vi "simpleReadWrite.vi"() -> ()   [LabVIEW 2015, in "labOpenShowVar.lvlib"]
uses:
  <vilib>/Platform/TimedLoop/XDataNode/timing_clust.ctl
  <vilib>/Platform/TimedLoop/XDataNode/nitl_modes.ctl
  <vilib>/Platform/TimedLoop/XDataNode/wakeup.ctl
  <vilib>/Platform/TimedLoop/XDataNode/XDataNode.xnode
  labOpenShowVar.lvlib
  <vilib>/Platform/TimedLoop/XDataNode/XDNodeRunTimeDep.lvlib
panel:
  in  "id":u16=1
  in  "写入":bool
  in  "value":string
  out "data":string
  in  "var":string="aaa"
  in  "停止":bool
  in  "ip":string="172.31.1.147"
  # "简单的变量读写"
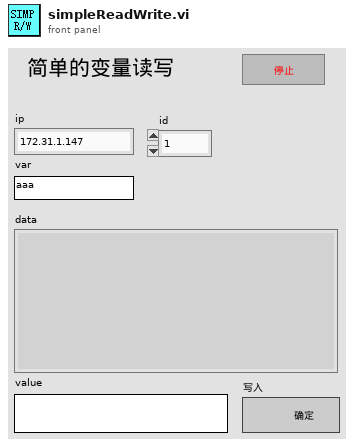
[diagram p1: front panel]
types:
  T1 = typedef "XDNodeRunTimeDep.lvlib/timing_clust.ctl" = cluster{"Expected End [f-1]":u64, "Actual End [f-1]":u64, "Finished Late? [f-1]":bool, "Expected End [i-1]":u64, "Actual End [i-1]":u64, "Finished Late? [i-1]":bool, "Expected Start [i]":u64, "Actual Start [i]":u64, "Expected Start [f]":u64, "Actual Start [f]":u64, "Source Name":string, "Structure Name":string, "Period":i64, "Deadline":i64, "Offset":i64, "Start":i64, "Priority":i32, "Timeout":i32, "Mode":T2, "Wakeup Reason":T3, "Error":errorcluster, "Source Type":string, "Secondary Source Type":string, "Global End Time":u64, "Global Start Time":u64, "Frame Duration":u64, "Iteration Duration":u64, "Assigned CPU":i32, "I/O Scan Engine Mode":u32}
  T2 = typedef "XDNodeRunTimeDep.lvlib/nitl_modes.ctl" = enum32{"No Change", "Process missed periods, maintain original phase", "Discard missed periods, maintain original phase", "Process missed periods, ignore original phase", "Discard missed periods, ignore original phase"}
  T3 = typedef "XDNodeRunTimeDep.lvlib/wakeup.ctl" = enum32{"Normal", "Aborted", "Asynchronous wakeup", "Timing source error", "Timed loop error", "Timeout"}
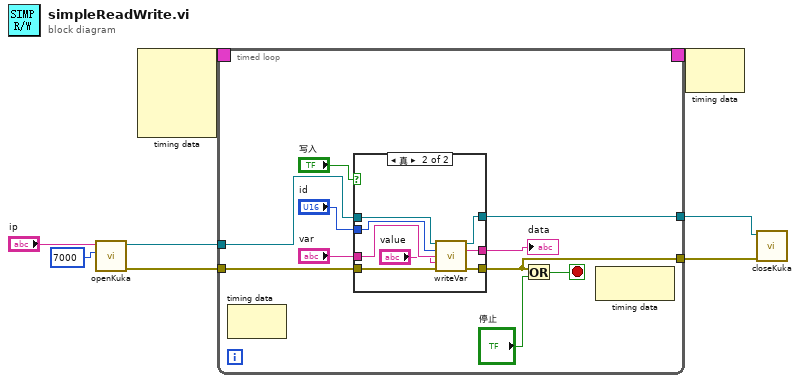
[diagram p0: block diagram]
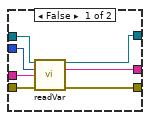
[diagram p2: hidden frame]
diagram:
  n1 = call "openKuka.vi"("远程端口或服务名称"=u16 7000, "地址"="ip") -> ("错误输出"=w5:errorcluster, "TCP网络连接输出"=w6:refnum<k5>)  [unwired: 8 in]
  n2 = node-c288() -> (w4:T1)  [unwired: 4 in]
  n3 = timed-loop {
    tunnel: w6 -> [w15]
    tunnel: w5 -> [w14]
    timing: w4 -> [_]
    timing-out: [_] -> w3
    tunnel: [w13] -> w2
    tunnel: [w10] -> w1
    stop <- w11 stop-if-true
    n4 = node-c288() -> ()  [unwired: 1 in, 1 out]
    n5 = case shown="真" "写入" {
      tunnel: "id" -> [w22 w32]
      tunnel: "var" -> [w21 w31]
      tunnel: w15 -> [w25 w33]
      tunnel: w14 -> [w24 w30]
      tunnel: [w23 w28] -> w13
      tunnel: [w20 w27] -> w10
      tunnel: [w19 w26] -> w9
      frame False {
        n6 = call "readVar.vi"("TCP网络连接输入"=w25, "id"=w22, "var"=w21, "错误输入（无错误）"=w24) -> ("TCP网络连接输出"=w23:refnum<k5>, "data out"=w19:string, "错误输出"=w20:errorcluster)  [unwired: 9 in]
      }
      frame True {
        n7 = call "writeVar.vi"("TCP网络连接输入"=w33, "id"=w32, "var"=w31, "val"="value", "错误输入（无错误）"=w30) -> ("TCP网络连接输出"=w28:refnum<k5>, "data out"=w26:string, "错误输出"=w27:errorcluster)  [unwired: 8 in]
      }
    }
    "data" <- w9
    n8 = Or(x=w10, y="停止") -> (x .or. y?=w11:bool)
    n9 = node-c288() -> ()  [unwired: 1 in, 1 out]
  }
  n10 = node-c288(w3) -> ()  [unwired: 1 out]
  n11 = call "closeKuka.vi"("错误输入（无错误）"=w1, "TCP网络连接输入"=w2) -> ()  [unwired: 10 in]
